vi "TranslateMe.vi"() -> ()   [LabVIEW 2017]
panel:
  out "Current Date and Time":string caption="Current Date or Time"
  in  "Date and Time":u16(ring) items=["Show Localized Time", "Show Localized Date"]
  in  "Show Dialog":bool caption="Show Localized Dialog"
  in  "Language ListBox":i32(listbox) caption="Language"
  out "Data.Display":dbl(graph) caption="Incoming Data"
  out "Error":bool
  in  "CustomControl.Increment":bool caption="Increment"
  out "Count":dbl
  in  "Exit":bool
  # "This VI is used to test translation"
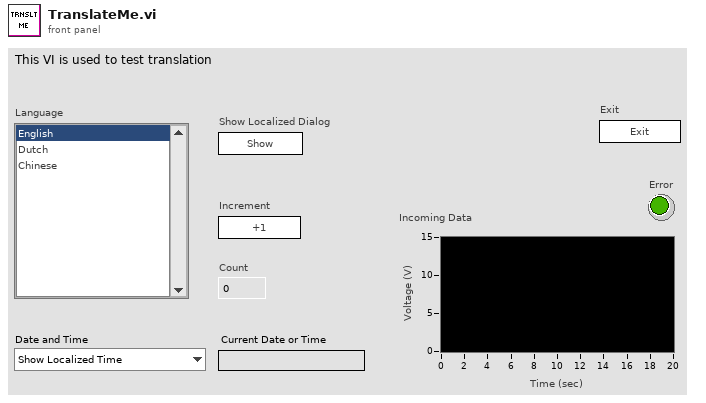
[diagram p1: front panel]
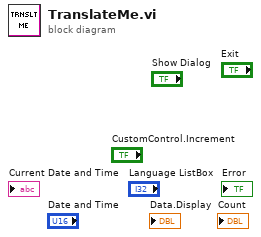
[diagram p0: block diagram]
diagram:
